vi "Create Connections.vi"(8 "error in (no error)":errorcluster, 11 "RT Data Cluster in":T1={"Timekeeper hdl"="", "clkDisc session"=variant, "Compiled Data"={"SyncMod?"=FALSE, "SyncMod"="", "ConnectionSettings"={"Mode"=enum."Generate sample clock", "pxitrig"=FALSE, "pfi0"=FALSE, "pfi1"=FALSE, "pfi2"=FALSE, "External Pin"=enum."PFI0", "Routes"=[]}, "TimeKeeper"="", "ScanOffset(%)"=0.0, "StartDelay(s)"=0, "Time Ref Settings"={"Time Reference"=enum."GPS", "Priority 1"=0, "Priority 2"=0, "IRIG type"=enum."IRIGB AM", "Terminal"="", "PPSSetTime"=FALSE, "Start Time"=timestamp(0 s since 1904-01-01)}, "FIFO Locations"={"BoardTime"=[], "Status"=[]}}, "OutputsData"=[], "OutputsFIFO"=refnum, "Scan Period"=0, "Timekeeper type"=enum."6683", "SyncMod type"=enum."6683", "SyncMod hdl"="", "Custom Device Name"=""} {"Compiled Data"."Time Ref Settings"."Priority 2" min=0 max=255; "Compiled Data"."Time Ref Settings"."Priority 1" min=0 max=255}) -> (0 "error out":errorcluster, 3 "RT Data Cluster out":T1={"Timekeeper hdl"="", "clkDisc session"=variant, "Compiled Data"={"SyncMod?"=FALSE, "SyncMod"="", "ConnectionSettings"={"Mode"=enum."Generate sample clock", "pxitrig"=FALSE, "pfi0"=FALSE, "pfi1"=FALSE, "pfi2"=FALSE, "External Pin"=enum."PFI0", "Routes"=[]}, "TimeKeeper"="", "ScanOffset(%)"=0.0, "StartDelay(s)"=0, "Time Ref Settings"={"Time Reference"=enum."GPS", "Priority 1"=0, "Priority 2"=0, "IRIG type"=enum."IRIGB AM", "Terminal"="", "PPSSetTime"=FALSE, "Start Time"=timestamp(0 s since 1904-01-01)}, "FIFO Locations"={"BoardTime"=[], "Status"=[]}}, "OutputsData"=[], "OutputsFIFO"=refnum, "Scan Period"=0, "Timekeeper type"=enum."6683", "SyncMod type"=enum."6683", "SyncMod hdl"="", "Custom Device Name"=""} {"Compiled Data"."Time Ref Settings"."Priority 2" min=0 max=255; "Compiled Data"."Time Ref Settings"."Priority 1" min=0 max=255})   [LabVIEW 2020, in "NI Synchronization Engine.lvlib"]
uses:
  NI Synchronization Engine.lvlib
  RT Data Cluster.ctl
  mdevClkDisc.llb/_clkDisc_session.ctl
  Shared/Compiled Data.ctl
  Shared/Connection Settings.ctl
  Shared/Mode.ctl
  Shared/External Pin.ctl
  Shared/Routes.ctl
  Shared/Route.ctl
  Shared/Time Ref Settings.ctl
  Shared/Time Reference.ctl
  Shared/IRIG Type.ctl
  timekeeper type.ctl
  Timekeeper Route Pin.ctl
  <instrlib>/niSync/niSync.llb/niSync Create Clock (Frequency).vi
  Shared/NI Synchronization Shared.lvlib
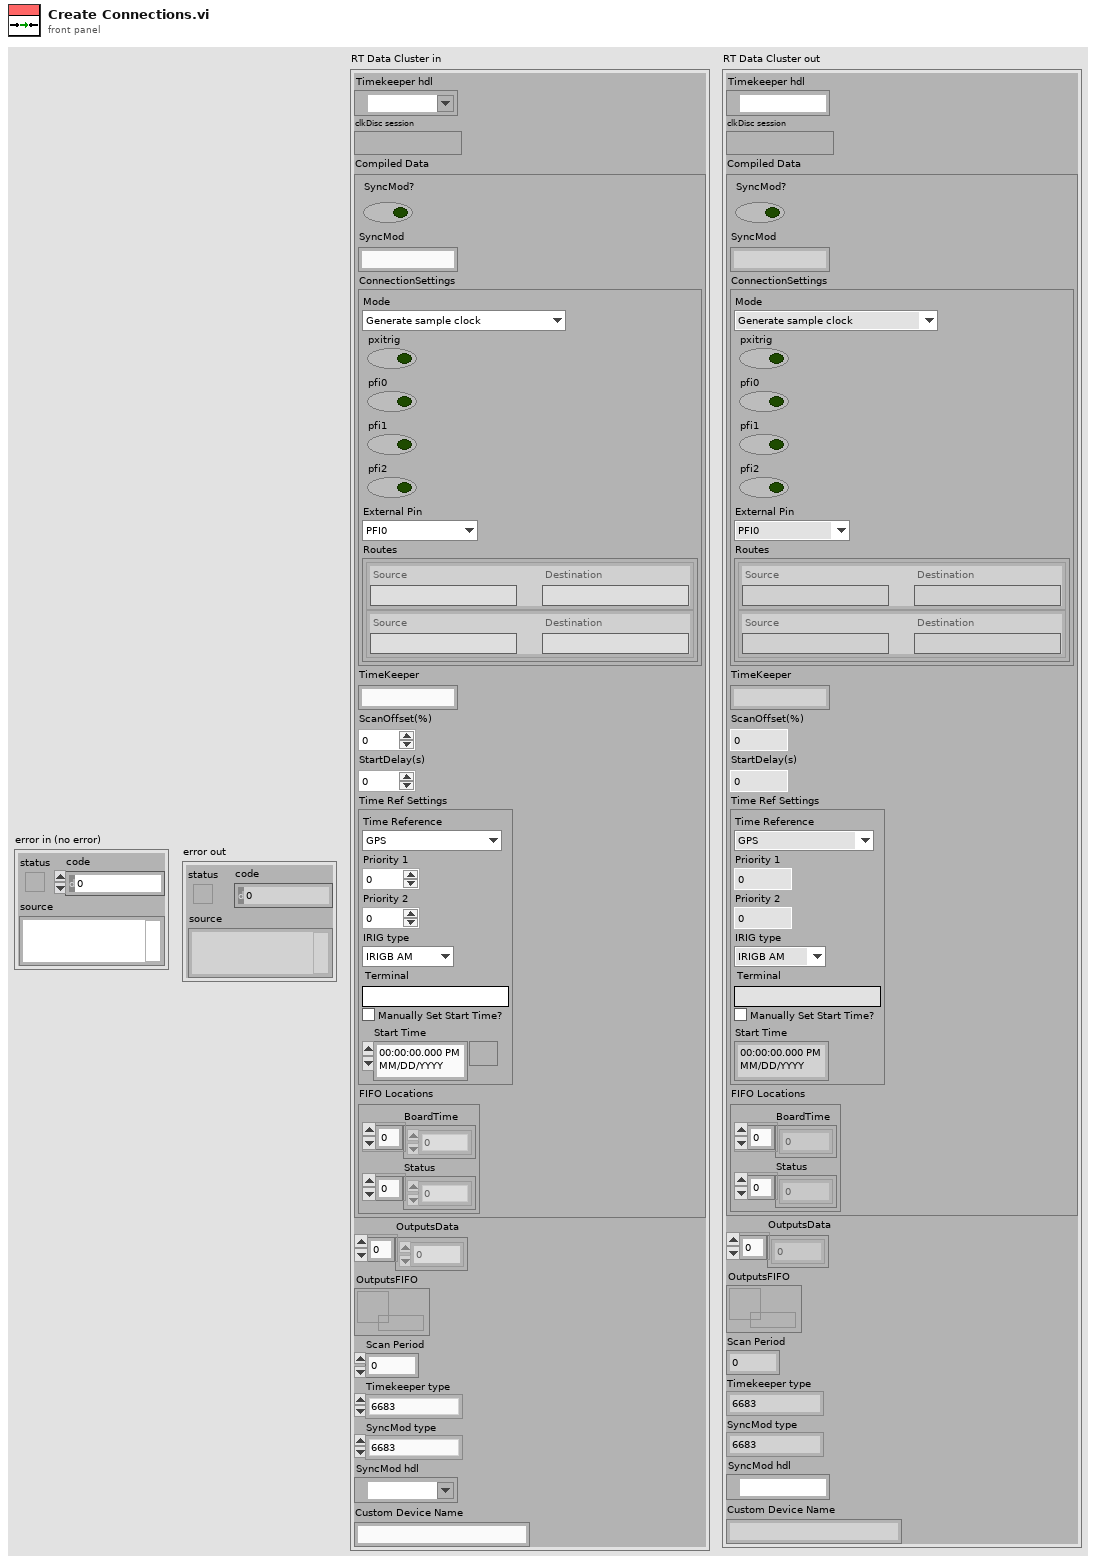
[diagram p1: front panel]
types:
  T1 = typedef "NI Synchronization Engine.lvlib/RT Data Cluster.ctl" = cluster{"Timekeeper hdl":refnum<k15>, "clkDisc session":T2, "Compiled Data":T3, "OutputsData":dbl[], "OutputsFIFO":refnum<k33>, "Scan Period":u32, "Timekeeper type":T12, "SyncMod type":T12, "SyncMod hdl":refnum<k15>, "Custom Device Name":string}
  T2 = typedef "_clkDisc_session.ctl" = variant
  T3 = typedef "NI Synchronization Shared.lvlib/Compiled Data.ctl" = cluster{"SyncMod?":bool, "SyncMod":string, "ConnectionSettings":T4, "TimeKeeper":string, "ScanOffset(%)":dbl, "StartDelay(s)":u16, "Time Ref Settings":T9, "FIFO Locations":cluster{"BoardTime":i32[], "Status":i32[]}}
  T4 = typedef "NI Synchronization Shared.lvlib/Connection Settings.ctl" = cluster{"Mode":T5, "pxitrig":bool, "pfi0":bool, "pfi1":bool, "pfi2":bool, "External Pin":T6, "Routes":T7}
  T5 = typedef "NI Synchronization Shared.lvlib/Mode.ctl" = enum16{"Generate sample clock", "Route sample clock out of chassis", "Route sample clock into chassis", "Custom routes"}
  T6 = typedef "NI Synchronization Shared.lvlib/External Pin.ctl" = enum16{"PFI0", "PFI1", "PFI2"}
  T7 = typedef "NI Synchronization Shared.lvlib/Routes.ctl" = T8[]
  T8 = typedef "NI Synchronization Shared.lvlib/Route.ctl" = cluster{"Source":string, "Destination":string}
  T9 = typedef "NI Synchronization Shared.lvlib/Time Ref Settings.ctl" = cluster{"Time Reference":T10, "Priority 1":i32, "Priority 2":i32, "IRIG type":T11, "Terminal":string, "PPSSetTime":bool, "Start Time":timestamp}
  T10 = typedef "NI Synchronization Shared.lvlib/Time Reference.ctl" = enum16{"GPS", "IRIG", "PPS", "1588 Ordinary Clock", "802.1AS", "PXI Chassis Clock", "Free Running (Internal)"}
  T11 = typedef "NI Synchronization Shared.lvlib/IRIG Type.ctl" = enum16{"IRIGB DC", "IRIGB AM"}
  T12 = typedef "NI Synchronization Engine.lvlib/timekeeper type.ctl" = enum16{"6683", "6683H", "6682", "6682H", "non-timekeeper", "timekeeper"}
  T13 = typedef "NI Synchronization Engine.lvlib/Timekeeper Route Pin.ctl" = enum16{"TTL0", "PFI0", "PFI1", "PFI2", "PXI_Clk10", "PXI_Clk10_In", "BoardClk", "ClkOut", "Oscillator"}
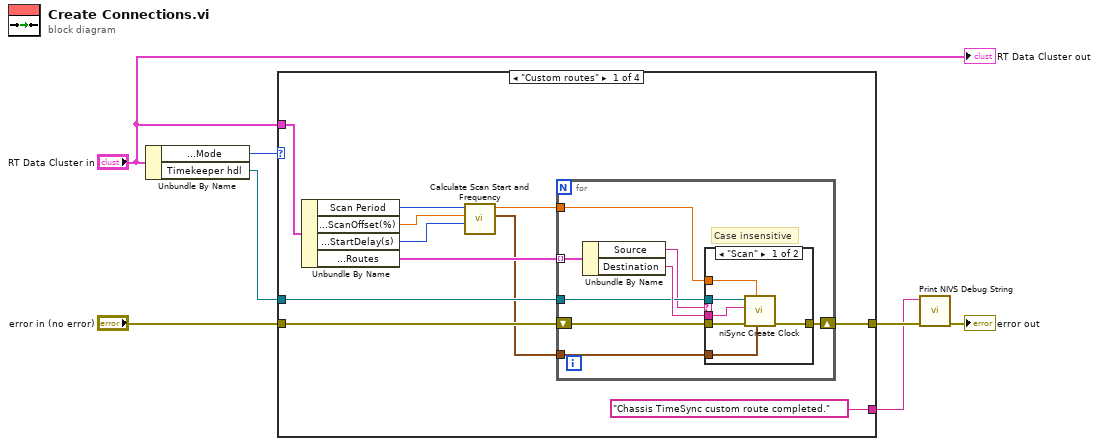
[diagram p0: block diagram]
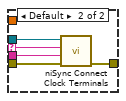
[diagram p2: hidden frame]
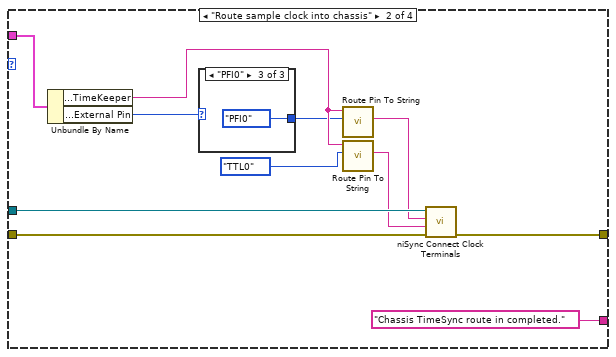
[diagram p3: hidden frame]
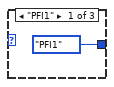
[diagram p4: hidden frame]
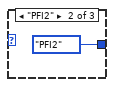
[diagram p5: hidden frame]
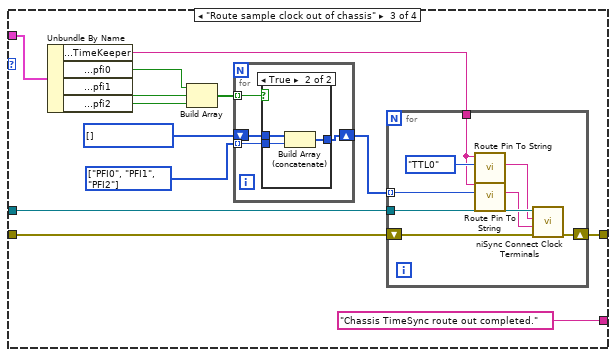
[diagram p6: hidden frame]
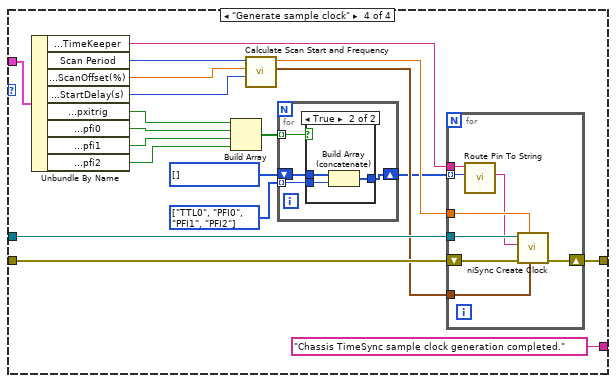
[diagram p8: hidden frame]
diagram:
  n1 = Unbundle By Name("RT Data Cluster in") -> ("Compiled Data.ConnectionSettings.Mode"=w7:T5, "Timekeeper hdl"=w6:refnum<k15>)
  n2 = case shown="\"Custom routes\"" w7 {
    tunnel: "error in (no error)" -> [w17 w42 w62 w96]
    tunnel: w6 -> [w13 w41 w61 w98]
    tunnel: "RT Data Cluster in" -> [w18 w48 w64 w95]
    tunnel: [w15 w46 w63 w99] -> w3
    tunnel: ["Chassis TimeSync custom route completed." "Chassis TimeSync route in completed." "Chassis TimeSync route out completed." "Chassis TimeSync sample clock generation completed."] -> w1
    frame "Custom routes" {
      n3 = Unbundle By Name(w18) -> ("Scan Period"=w12:u32, "Compiled Data.ScanOffset(%)"=w11:dbl, "Compiled Data.StartDelay(s)"=w10:u16, "Compiled Data.ConnectionSettings.Routes"=w16:T7)
      n4 = call "Calculate Scan Start and Frequency.vi"("Start delay (s)"=w10, "Start offset (fraction)"=w11, "Scan Period (uS)"=w12) -> ("Start time"=w8:timestamp, "Frequency"=w9:dbl)  [unwired: 7 in]
      n5 = for {
        shift-right: [w23] -> w15
        shift-left: w17 -> [w26]
        tunnel: w16 -> [w25] mode=indexing
        tunnel: w13 -> [w22]
        tunnel: w9 -> [w20]
        tunnel: w8 -> [w19]
        # "Case insensitive"
        n6 = Unbundle By Name(w25) -> ("Source"=w21:string, "Destination"=w24:string)
        n7 = case shown="\"Scan\"" w21 {
          selector: w21 -> [_ w33]
          tunnel: w26 -> [w32 w37]
          tunnel: w24 -> [w27 w36]
          tunnel: [w31 w35] -> w23
          tunnel: w22 -> [w30 w34]
          tunnel: w20 -> [w29 _]
          tunnel: w19 -> [w28 _]
          frame "Scan" {
            n8 = call-poly <instrlib>:"niSync Create Clock.vi"("start time"=w28, "frequency"=w29, "error in (no error)"=w32, "terminal"=w27, "instrument handle"=w30) -> ("error out"=w31:errorcluster)  [unwired: 3 in, 3 out]
          }
          frame Default {
            n9 = call <instrlib>:"niSync Connect Clock Terminals.vi"("error in (no error)"=w37, "destination terminal"=w36, "source terminal"=w33, "instrument handle"=w34) -> ("error out"=w35:errorcluster)  [unwired: 6 in, 1 out]
          }
        }
      }
    }
    frame "Route sample clock into chassis" {
      n10 = Unbundle By Name(w48) -> ("Compiled Data.TimeKeeper"=w45:string, "Compiled Data.ConnectionSettings.External Pin"=w47:T6)
      n11 = case shown="\"PFI0\"" w47 {
        tunnel: [Timekeeper_Route_Pin."PFI1" ("Pin") Timekeeper_Route_Pin."PFI2" ("Pin") Timekeeper_Route_Pin."PFI0" ("Pin")] -> w43
        frame "PFI1" {
        }
        frame "PFI2" {
        }
        frame "PFI0" {
        }
      }
      n12 = call "Route Pin To String.vi"("Pin"=w43, "Module"=w45) -> ("String"=w40:string)  [unwired: 9 in]
      n13 = call "Route Pin To String.vi"("Pin"=Timekeeper_Route_Pin."TTL0", "Module"=w45) -> ("String"=w39:string)  [unwired: 9 in]
      n14 = call <instrlib>:"niSync Connect Clock Terminals.vi"("error in (no error)"=w42, "destination terminal"=w39, "source terminal"=w40, "instrument handle"=w41) -> ("error out"=w46:errorcluster)  [unwired: 6 in, 1 out]
    }
    frame "Route sample clock out of chassis" {
      w54 = T13[] [enum."PFI0", enum."PFI1", enum."PFI2"] items=["TTL0", "PFI0", "PFI1", "PFI2", "PXI_Clk10", "PXI_Clk10_In", "BoardClk", "ClkOut", "Oscillator"]
      w55 = T13[] [] items=["TTL0", "PFI0", "PFI1", "PFI2", "PXI_Clk10", "PXI_Clk10_In", "BoardClk", "ClkOut", "Oscillator"]
      n15 = Unbundle By Name(w64) -> ("Compiled Data.TimeKeeper"=w60:string, "Compiled Data.ConnectionSettings.pfi0"=w59:bool, "Compiled Data.ConnectionSettings.pfi1"=w58:bool, "Compiled Data.ConnectionSettings.pfi2"=w57:bool)
      n16 = Build Array(w59, w58, w57) -> (w56:bool[])
      n17 = for {
        tunnel: w56 -> [w68] mode=indexing
        shift-right: [w65] -> w53
        shift-left: w55 -> [w67]
        tunnel: w54 -> [w66] mode=indexing
        n18 = case shown="True" w68 {
          tunnel: w67 -> [w69 w72]
          tunnel: w66 -> [_ w71]
          tunnel: [w69 w70] -> w65
          frame False {
          }
          frame True {
            n19 = Build Array (concatenate)(w72, w71) -> (w70:T13[])
          }
        }
      }
      n20 = for {
        tunnel: w61 -> [w78]
        shift-right: [w80] -> w63
        shift-left: w62 -> [w79]
        tunnel: w60 -> [w75]
        tunnel: w53 -> [w73] mode=indexing
        n21 = call "Route Pin To String.vi"("Pin"=Timekeeper_Route_Pin."TTL0", "Module"=w75) -> ("String"=w77:string)  [unwired: 9 in]
        n22 = call "Route Pin To String.vi"("Pin"=w73, "Module"=w75) -> ("String"=w74:string)  [unwired: 9 in]
        n23 = call <instrlib>:"niSync Connect Clock Terminals.vi"("error in (no error)"=w79, "destination terminal"=w74, "source terminal"=w77, "instrument handle"=w78) -> ("error out"=w80:errorcluster)  [unwired: 6 in, 1 out]
      }
    }
    frame "Generate sample clock" {
      w87 = T13[] [enum."TTL0", enum."PFI0", enum."PFI1", enum."PFI2"] items=["TTL0", "PFI0", "PFI1", "PFI2", "PXI_Clk10", "PXI_Clk10_In", "BoardClk", "ClkOut", "Oscillator"]
      w88 = T13[] [] items=["TTL0", "PFI0", "PFI1", "PFI2", "PXI_Clk10", "PXI_Clk10_In", "BoardClk", "ClkOut", "Oscillator"]
      n24 = Unbundle By Name(w95) -> ("Compiled Data.TimeKeeper"=w85:string, "Scan Period"=w94:u32, "Compiled Data.ScanOffset(%)"=w93:dbl, "Compiled Data.StartDelay(s)"=w92:u16, "Compiled Data.ConnectionSettings.pxitrig"=w84:bool, "Compiled Data.ConnectionSettings.pfi0"=w83:bool, "Compiled Data.ConnectionSettings.pfi1"=w82:bool, "Compiled Data.ConnectionSettings.pfi2"=w81:bool)
      n25 = Build Array(w84, w83, w82, w81) -> (w89:bool[])
      n26 = call "Calculate Scan Start and Frequency.vi"("Start delay (s)"=w92, "Start offset (fraction)"=w93, "Scan Period (uS)"=w94) -> ("Start time"=w90:timestamp, "Frequency"=w91:dbl)  [unwired: 7 in]
      n27 = for {
        tunnel: w89 -> [w103] mode=indexing
        shift-right: [w100] -> w86
        shift-left: w88 -> [w102]
        tunnel: w87 -> [w101] mode=indexing
        n28 = case shown="True" w103 {
          tunnel: w102 -> [w104 w107]
          tunnel: w101 -> [_ w106]
          tunnel: [w104 w105] -> w100
          frame False {
          }
          frame True {
            n29 = Build Array (concatenate)(w107, w106) -> (w105:T13[])
          }
        }
      }
      n30 = for {
        shift-right: [w114] -> w99
        shift-left: w96 -> [w115]
        tunnel: w98 -> [w113]
        tunnel: w91 -> [w112]
        tunnel: w90 -> [w111]
        tunnel: w86 -> [w110] mode=indexing
        tunnel: w85 -> [w108]
        n31 = call "Route Pin To String.vi"("Pin"=w110, "Module"=w108) -> ("String"=w109:string)  [unwired: 9 in]
        n32 = call-poly <instrlib>:"niSync Create Clock.vi"("start time"=w111, "frequency"=w112, "error in (no error)"=w115, "terminal"=w109, "instrument handle"=w113) -> ("error out"=w114:errorcluster)  [unwired: 3 in, 3 out]
      }
    }
  }
  n33 = call "Print NIVS Debug String.vi"("error in (no error)"=w3, "Debug String"=w1) -> ("error out"=→"error out":errorcluster)  [unwired: 8 in]
  "RT Data Cluster out" <- "RT Data Cluster in"
